vi "eDyno NVH Accel Simulator.vi"() -> ()   [LabVIEW 2026]
doc: "eDyno NVH accelerometer SIMULATOR - analog output only (PXIe-4468 AO0).\n\nContinuously generates, with NI-DAQmx and regeneration disabled, a voltage that emulates a PCB 356A15 ICP accelerometer (one axis, Sensitivity mV/g, default 100) on an e-bike drive unit on the eDyno. Acquisition and analysis are deliberately NOT here: run them in a separate VI on any AI channel wired to AO0 (with IEPE excitation OFF on that channel - never drive an AO into an IEPE-powered input).\n\nSpeed: constant, or a linear run-up when Speed Profile / Run-up Enabled is ON; every order tracks speed. Switch faults on live in Fault Injection:\n1) Imbalance (1x order, grows with rpm^2) / Misalignment (2x order)\n2) Bearing outer-race defect (impacts at BPFO ringing the housing resonance: crest factor and kurtosis rise, BPFO-spaced lines around the resonance)\n3) Motor torque ripple (6 x pole pairs order) and inverter PWM carrier with +/-2fe sidebands.\n\nFault Frequencies shows where each fault should appear at the current speed (the answer key for the analysis VI).\n\nTiming: the AO buffer holds 3 blocks and DAQmx Write blocks when it is full, so the loop is paced by the hardware clock and a front-panel change reaches the output within about 3 x (Samples per Block / Sample Rate)."
uses:
  <vilib>/xnet/xnet.llb/XNET Mode.ctl
  <extravilib>/ChannelInstances/Messenger-bool/Read With Abort.vi
  <extravilib>/ChannelInstances/Messenger-bool/Write With Abort.vi
  <vilib>/xnet/xnet.llb/XNET Create Session (Generic).vi
  <extravilib>/ChannelInstances/Messenger-bool/Instantiate.vi
  <extravilib>/ChannelInstances/Messenger-bool/Endpoint.vi
  <vilib>/xnet/xnet.llb/XNET Write (Signal Single-point).vi
  <vilib>/DAQmx/miscellaneous.llb/DAQmx Fill In Error Info.vi
  <extravilib>/ChannelInstances/Messenger-bool.lvlib
  <resource>/objmgr/xnet.rc
panel:
  out "Load Torque (Nm)":dbl
  in  "Acc_Out":tag="DSA_4468/ao0"
  out "Simulated Acceleration (g)":dbl[](graph)
  out "Fault Frequencies (Hz)":T1={"1x Shaft"=50.0, "2x Misalign"=100.0, "BPFO"=178.5, "Torque Ripple"=1200.0, "PWM Carrier"=16000.0}
  out "Shaft Speed (rpm)":dbl(knob)=3000.0 scale=0.0..5000.0
  in  "STOP":bool
  in  "Speed Profile":T2={"Run-up Enabled"=FALSE, "Constant Speed (rpm)"=3000.0, "Run-up Start (rpm)"=500.0, "Run-up End (rpm)"=4500.0, "Run-up Duration (s)"=30.0}
  in  "Sim Config":T3={"Sample Rate (Hz)"=51200.0, "Ref Speed (rpm)"=3000.0, "Baseline 1x (g)"=0.02, "Noise Floor (g rms)"=0.01, "BPFO Order"=3.57, "Resonance (Hz)"=3500.0, "Decay (ms)"=0.8, "Pole Pairs"=4.0, "PWM Carrier (Hz)"=16000.0}
  in  "Fault Injection":T4={"Imbalance ON"=FALSE, "Imbalance (g)"=0.5, "Misalignment ON"=FALSE, "Misalignment (g)"=0.2, "Bearing BPFO ON"=FALSE, "Bearing Impact (g)"=2.0, "Motor Ripple ON"=FALSE, "Torque Ripple (g)"=0.3, "PWM Noise ON"=FALSE, "PWM Level (g)"=0.05}
  in  "AO Range (V)":dbl=10.0
  in  "Sensitivity (mV/g)":dbl=1000.0
  in  "Samples per Block":i32=5120
  in  "Sample Rate (S/s)":dbl=51200.0
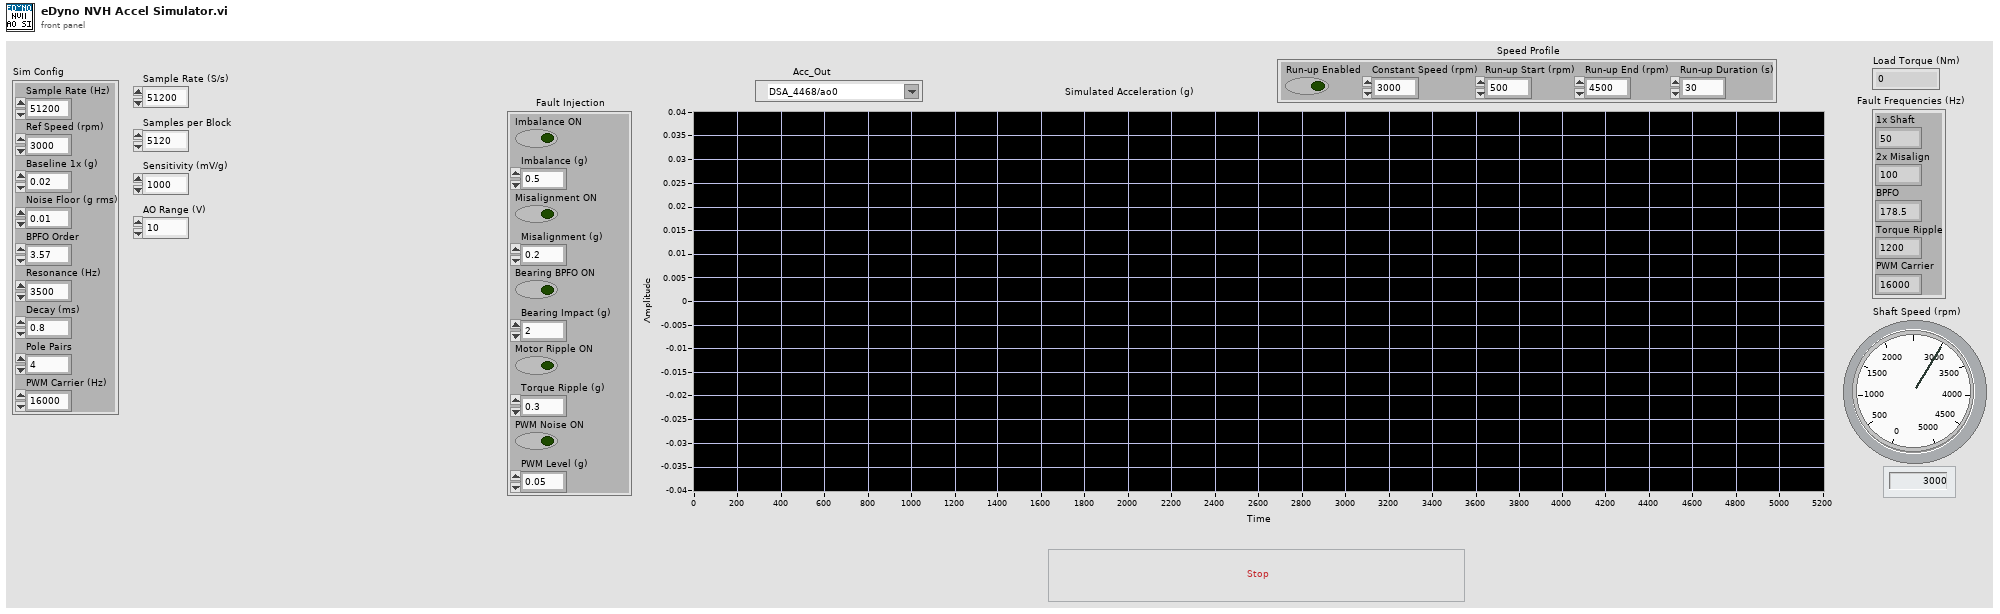
[diagram p1: front panel]
types:
  T1 = cluster{"1x Shaft":dbl, "2x Misalign":dbl, "BPFO":dbl, "Torque Ripple":dbl, "PWM Carrier":dbl}
  T2 = cluster{"Run-up Enabled":bool, "Constant Speed (rpm)":dbl, "Run-up Start (rpm)":dbl, "Run-up End (rpm)":dbl, "Run-up Duration (s)":dbl}
  T3 = cluster{"Sample Rate (Hz)":dbl, "Ref Speed (rpm)":dbl, "Baseline 1x (g)":dbl, "Noise Floor (g rms)":dbl, "BPFO Order":dbl, "Resonance (Hz)":dbl, "Decay (ms)":dbl, "Pole Pairs":dbl, "PWM Carrier (Hz)":dbl}
  T4 = cluster{"Imbalance ON":bool, "Imbalance (g)":dbl, "Misalignment ON":bool, "Misalignment (g)":dbl, "Bearing BPFO ON":bool, "Bearing Impact (g)":dbl, "Motor Ripple ON":bool, "Torque Ripple (g)":dbl, "PWM Noise ON":bool, "PWM Level (g)":dbl}
  T5 = typedef "XNET Mode.ctl" = u32
  T6 = cluster{"Fault Injection":cluster{"Imbalance ON":bool, "Imbalance (g)":dbl, "Misalignment ON":bool, "Misalignment (g)":dbl, "Bearing BPFO ON":bool, "Bearing Impact (g)":dbl, "Motor Ripple ON":bool, "Torque Ripple (g)":dbl, "PWM Noise ON":bool, "PWM Level (g)":dbl}, "Shaft Speed (rpm)":dbl, "Fault Frequencies (Hz)":cluster{"1x Shaft":dbl, "2x Misalign":dbl, "BPFO":dbl, "Torque Ripple":dbl, "PWM Carrier":dbl}, "Speed Profile":cluster{"Run-up Enabled":bool, "Constant Speed (rpm)":dbl, "Run-up Start (rpm)":dbl, "Run-up End (rpm)":dbl, "Run-up Duration (s)":dbl}, "Sim Config":cluster{"Sample Rate (Hz)":dbl, "Ref Speed (rpm)":dbl, "Baseline 1x (g)":dbl, "Noise Floor (g rms)":dbl, "BPFO Order":dbl, "Resonance (Hz)":dbl, "Decay (ms)":dbl, "Pole Pairs":dbl, "PWM Carrier (Hz)":dbl}, "AO_Loop_Count":i32, "Accel (g)":dbl[]}
  T7 = typedef "Messenger-bool.lvlib/))Channel.ctl" = refnum<queue>
  T8 = cluster{"Speed Act (rpm)":dbl, "Torque (Nm)":dbl, "Test Step":dbl, "Seq State":dbl, "Block Counter":dbl, "Alive Counter":dbl}
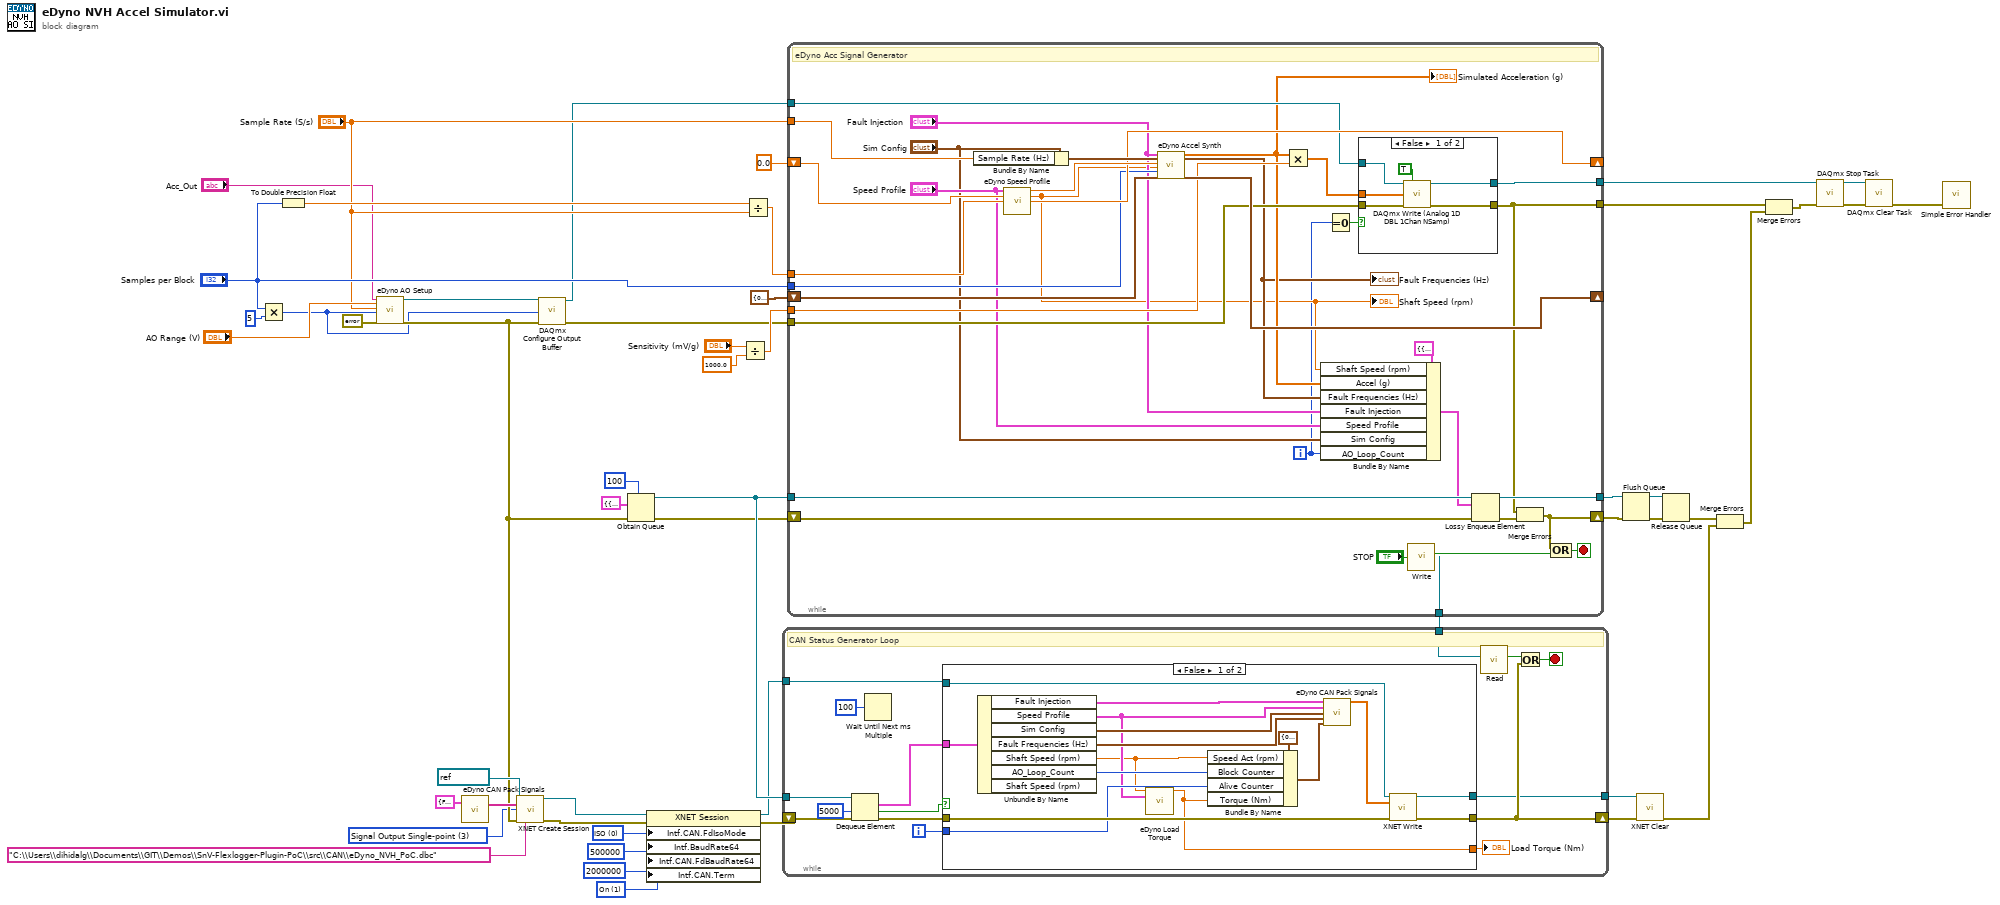
[diagram p0: block diagram]
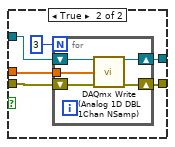
[diagram p2: hidden frame]
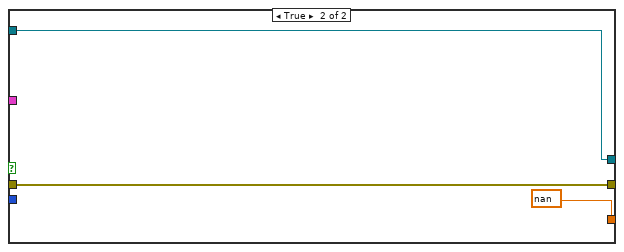
[diagram p3: hidden frame]
diagram:
  w10 = u32 1 items=["Off", "On"] ("Interface:CAN:Termination")
  w13 = u32 0 items=["ISO", "Non ISO", "ISO Legacy"] ("Interface:CAN:FD ISO Mode")
  w22 = T5 3 items=["Signal Input Single-point", "Signal Input Waveform", "Signal Input XY", "Signal Output Single-point", "Signal Output Waveform", "Signal Output XY", "Frame Input Stream", "Frame Input Queued", "Frame Input Single-point", "Frame Output Stream", "Frame Output Queued", "Frame Output Single-point", "Conversion"] ("mode")
  n1 = Multiply(x="Samples per Block", y=5 ("3 blocks")) -> (x*y=w2:i32)
  n2 = To Double Precision Float(number="Samples per Block") -> (double precision float=w43:dbl)
  n3 = call "eDyno AO Setup.vi"("physical channels"="Acc_Out", "AO Range (V)"="AO Range (V)", "Sample Rate (S/s)"="Sample Rate (S/s)", "Buffer Samples"=w2, "error in"=errorcluster {"status"=FALSE, "code"=0, "source"=""} ("no error")) -> ("task out"=w4:refnum<k21>, "error out"=w25:errorcluster)  [unwired: 13 in]
  n4 = call "eDyno CAN Pack Signals.vi"("Fault Injection"=T4 {"Imbalance ON"=FALSE, "Imbalance (g)"=0.5, "Misalignment ON"=FALSE, "Misalignment (g)"=0.2, "Bearing BPFO ON"=FALSE, "Bearing Impact (g)"=2.0, "Motor Ripple ON"=FALSE, "Torque Ripple (g)"=0.3, "PWM Noise ON"=FALSE, "PWM Level (g)"=0.05}) -> ("Signal List"=w27:string[])  [unwired: 12 in, 2 out]
  n5 = call-poly <vilib>:"XNET Create Session.vi"("list (empty)"=w27, "mode"=w22, "interface"=refnum<k21> "CAN1", "error in (no error)"=w25, "database (:memory:)"="C:\\Users\\dihidalg\\Documents\\GIT\\Demos\\SnV-Flexlogger-Plugin-PoC\\src\\CAN\\eDyno_NVH_PoC.dbc") -> ("session out"=w15:refnum<k21>, "error out"=w24:errorcluster)  [unwired: 9 in]
  n6 = call <vilib>:"DAQmx Configure Output Buffer.vi"("task/channels in"=w4, "buffer size (in samples per channel)"=w2, "error in"=w25) -> ("task out"=w3:refnum<k21>, "error out"=w5:errorcluster)  [unwired: 11 in]
  n7 = Obtain Queue(max queue size (-1, unlimited)=100, element data type=T6 {"Fault Injection"={"Imbalance ON"=FALSE, "Imbalance (g)"=0.5, "Misalignment ON"=FALSE, "Misalignment (g)"=0.2, "Bearing BPFO ON"=FALSE, "Bearing Impact (g)"=2.0, "Motor Ripple ON"=FALSE, "Torque Ripple (g)"=0.3, "PWM Noise ON"=FALSE, "PWM Level (g)"=0.05}, "Shaft Speed (rpm)"=0.0, "Fault Frequencies (Hz)"={"1x Shaft"=0.0, "2x Misalign"=0.0, "BPFO"=0.0, "Torque Ripple"=0.0, "PWM Carrier"=0.0}, "Speed Profile"={"Run-up Enabled"=TRUE, "Constant Speed (rpm)"=3000.0, "Run-up Start (rpm)"=500.0, "Run-up End (rpm)"=4500.0, "Run-up Duration (s)"=30.0}, "Sim Config"={"Sample Rate (Hz)"=51200.0, "Ref Speed (rpm)"=3000.0, "Baseline 1x (g)"=0.02, "Noise Floor (g rms)"=0.01, "BPFO Order"=3.57, "Resonance (Hz)"=3500.0, "Decay (ms)"=0.8, "Pole Pairs"=4.0, "PWM Carrier (Hz)"=16000.0}, "AO_Loop_Count"=0, "Accel (g)"=[]} ("output cluster"), error in (no error)=w25) -> (queue out=w33:refnum<queue>, error out=w31:errorcluster)  [unwired: 2 in, 1 out]
  n8 = property class="XNET Session"(reference=w15, error in=w24, "Intf.CAN.FdIsoMode"=w13, "Intf.BaudRate64"=u64 500000 ("Interface:64bit Baud Rate"), "Intf.CAN.FdBaudRate64"=u64 2000000 ("Interface:CAN:64bit FD Baud Rate"), "Intf.CAN.Term"=w10) -> (reference out=w14:refnum<k21>, error out=w16:errorcluster)
  n9 = Divide(x="Sensitivity (mV/g)", y=1000.0 ("mV per V")) -> (x/y=w42:dbl)
  n10 = Divide(x=w43, y="Sample Rate (S/s)") -> (x/y=w44:dbl)
  n11 = while {
    tunnel: "Sample Rate (S/s)" -> [w71]
    tunnel: "Samples per Block" -> [w72]
    shift-right: [w76] -> _
    shift-left: 0.0 ("run-up t0 (s)") -> [w75]
    shift-right: [w81] -> _
    shift-left: cluster{"Shaft Rev":dbl, "Sample Index":dbl} {"Shaft Rev"=0.0, "Sample Index"=0.0} ("initial synth state") -> [w77]
    tunnel: w42 -> [w73]
    tunnel: w3 -> [w69]
    tunnel: w5 -> [w70]
    tunnel: w44 -> [w74]
    tunnel: [w83] -> w47
    tunnel: [w62] -> w48
    tunnel: w33 -> [w66]
    tunnel: [w63] -> w30
    tunnel: [w55] -> w21
    shift-right: [w61] -> w29
    shift-left: w31 -> [w65]
    i -> [w52]
    stop <- w84 stop-if-true
    # "eDyno Acc Signal Generator"
    n12 = Bundle By Name(cluster="Sim Config", "Sample Rate (Hz)"=w71) -> (w80:T3)
    n13 = call "eDyno Speed Profile.vi"("Speed Profile"="Speed Profile", "t in (s)"=w75, "Block Duration (s)"=w74) -> ("rpm start"=w79:dbl, "rpm end"=w54:dbl, "t out (s)"=w76:dbl)  [unwired: 10 in]
    "Shaft Speed (rpm)" <- w54
    n14 = call "eDyno Accel Synth.vi"("Fault Injection"="Fault Injection", "Sim Config"=w80, "rpm start"=w79, "rpm end"=w54, "Samples"=w72, "State in"=w77) -> ("Accel (g)"=w68:dbl[], "Fault Frequencies (Hz)"=w67:T1, "State out"=w81:cluster{"Shaft Rev":dbl, "Sample Index":dbl})  [unwired: 9 in, 2 out]
    "Fault Frequencies (Hz)" <- w67
    "Simulated Acceleration (g)" <- w68
    n15 = Multiply(x=w68, y=w73) -> (x*y=w82:dbl[])
    n16 = Bundle By Name(cluster=T6 {"Fault Injection"={"Imbalance ON"=FALSE, "Imbalance (g)"=0.5, "Misalignment ON"=FALSE, "Misalignment (g)"=0.2, "Bearing BPFO ON"=FALSE, "Bearing Impact (g)"=2.0, "Motor Ripple ON"=FALSE, "Torque Ripple (g)"=0.3, "PWM Noise ON"=FALSE, "PWM Level (g)"=0.05}, "Shaft Speed (rpm)"=0.0, "Fault Frequencies (Hz)"={"1x Shaft"=0.0, "2x Misalign"=0.0, "BPFO"=0.0, "Torque Ripple"=0.0, "PWM Carrier"=0.0}, "Speed Profile"={"Run-up Enabled"=TRUE, "Constant Speed (rpm)"=3000.0, "Run-up Start (rpm)"=500.0, "Run-up End (rpm)"=4500.0, "Run-up Duration (s)"=30.0}, "Sim Config"={"Sample Rate (Hz)"=51200.0, "Ref Speed (rpm)"=3000.0, "Baseline 1x (g)"=0.02, "Noise Floor (g rms)"=0.01, "BPFO Order"=3.57, "Resonance (Hz)"=3500.0, "Decay (ms)"=0.8, "Pole Pairs"=4.0, "PWM Carrier (Hz)"=16000.0}, "AO_Loop_Count"=0, "Accel (g)"=[]} ("output cluster"), "Shaft Speed (rpm)"=w54, "Accel (g)"=w68, "Fault Frequencies (Hz)"=w67, "Fault Injection"="Fault Injection", "Speed Profile"="Speed Profile", "Sim Config"="Sim Config", "AO_Loop_Count"=w52) -> (w56:T6)
    n17 = Equal To 0?(x=w52) -> (x = 0?=w53:bool)
    n18 = case shown="False" w53 {
      tunnel: [w90 w94] -> w83
      tunnel: w82 -> [w89 w92]
      tunnel: w70 -> [w88 w95]
      tunnel: w69 -> [w87 w96]
      tunnel: [w85 w93] -> w62
      frame False {
        n19 = call <vilib>:"DAQmx Write (Analog 1D DBL 1Chan NSamp).vi"("task/channels in"=w87, "auto start"=TRUE, "data"=w89, "error in"=w88) -> ("task out"=w90:refnum<k21>, "error out"=w85:errorcluster)  [unwired: 9 in, 1 out]
      }
      frame True {
        n20 = for {
          N: 3 -> [_]
          tunnel: w92 -> [w97]
          shift-right: [w99] -> w94
          shift-left: w96 -> [w101]
          shift-right: [w98] -> w93
          shift-left: w95 -> [w100]
          n21 = call <vilib>:"DAQmx Write (Analog 1D DBL 1Chan NSamp).vi"("task/channels in"=w101, "data"=w97, "error in"=w100) -> ("task out"=w99:refnum<k21>, "error out"=w98:errorcluster)  [unwired: 10 in, 1 out]
        }
      }
    }
    n22 = call <extravilib>:"Write.vi"("element"="STOP") -> ("channel"=w55:T7)  [unwired: 8 in, 2 out]
    n23 = Lossy Enqueue Element(queue=w66, element=w56, error in (no error)=w65) -> (queue out=w63:refnum<queue>, error out=w64:errorcluster)  [unwired: 2 out]
    n24 = Merge Errors(w62, w64) -> (w61:errorcluster)
    n25 = Compound Arithmetic op=OR(w61, "STOP") -> (w84:bool)
  }
  n26 = while {
    tunnel: w33 -> [w103]
    tunnel: w14 -> [w114]
    tunnel: w21 -> [w111]
    tunnel: [w107] -> w19
    shift-right: [w108] -> w20
    shift-left: w16 -> [w115]
    i -> [w112]
    stop <- w109 stop-if-true
    # "CAN Status Generator Loop"
    n27 = Dequeue Element(queue=w103, timeout in ms (-1)=5000, error in (no error)=w115) -> (element=w116:T6, timed out?=w104:bool, error out=w113:errorcluster)  [unwired: 1 out]
    n28 = Wait Until Next ms Multiple(millisecond multiple=u32 100) -> ()  [unwired: 1 out]
    n29 = case shown="False" w104 {
      tunnel: w116 -> [w132 _]
      tunnel: w114 -> [w128 w135]
      tunnel: w113 -> [w127 w134]
      tunnel: w112 -> [w123 _]
      tunnel: [w121 w134] -> w108
      tunnel: [w120 w135] -> w107
      tunnel: [w117 nan ("Load Torque (Nm)")] -> w102
      frame False {
        n30 = Unbundle By Name(w132) -> ("Fault Injection"=w131:T4, "Speed Profile"=w119:T2, "Sim Config"=w130:T3, "Fault Frequencies (Hz)"=w129:T1, "Shaft Speed (rpm)"=w118:dbl, "AO_Loop_Count"=w124:i32)  [unwired: 1 out]
        n31 = call "eDyno Load Torque.vi"("Speed (rpm)"=w118, "Speed Profile"=w119) -> ("Load Torque (Nm)"=w117:dbl)  [unwired: 13 in]
        n32 = Bundle By Name(cluster=T8 {"Speed Act (rpm)"=0.0, "Torque (Nm)"=0.0, "Test Step"=0.0, "Seq State"=0.0, "Block Counter"=0.0, "Alive Counter"=0.0} ("Status"), "Speed Act (rpm)"=w118, "Block Counter"=w124, "Alive Counter"=w123, "Torque (Nm)"=w117) -> (w125:T8)
        n33 = call "eDyno CAN Pack Signals.vi"("Fault Injection"=w131, "Speed Profile"=w119, "Sim Config"=w130, "Fault Frequencies (Hz)"=w129, "Status"=w125) -> ("Signal Values"=w122:dbl[])  [unwired: 8 in, 2 out]
        n34 = call-poly <vilib>:"XNET Write.vi"("session in"=w128, "data"=w122, "error in (no error)"=w127) -> ("session out"=w120:refnum<k21>, "error out"=w121:errorcluster)  [unwired: 11 in]
      }
      frame True {
      }
    }
    "Load Torque (Nm)" <- w102
    n35 = call <extravilib>:"Read.vi"("channel"=w111) -> ("element"=w110:bool)  [unwired: 8 in, 2 out]
    n36 = Or(x=w110, y=w108) -> (x .or. y?=w109:bool)
  }
  n37 = Flush Queue(queue=w30, error in (no error)=w29) -> (queue out=w35:refnum<queue>, error out=w8:errorcluster)  [unwired: 1 out]
  n38 = call <vilib>:"XNET Clear.vi"("session in"=w19, "error in (no error)"=w20) -> ("error out"=w17:errorcluster)  [unwired: 13 in]
  n39 = Release Queue(queue=w35, error in (no error)=w8) -> (error out=w7:errorcluster)  [unwired: 1 in, 2 out]
  n40 = Merge Errors(w7, w17) -> (w6:errorcluster)
  n41 = Merge Errors(w48, w6) -> (w28:errorcluster)
  n42 = call <vilib>:"DAQmx Stop Task.vi"("task/channels in"=w47, "error in"=w28) -> ("task out"=w49:refnum<k21>, "error out"=w50:errorcluster)  [unwired: 12 in]
  n43 = call <vilib>:"DAQmx Clear Task.vi"("task in"=w49, "error in"=w50) -> ("error out"=w51:errorcluster)  [unwired: 13 in]
  n44 = call <vilib>:"Simple Error Handler.vi"("error in (no error)"=w51) -> ()  [unwired: 4 in, 5 out]
